vi "GPIB_SR400_A.vi"(11 "N per point":i32=1) -> (0 "A Gate":dbl[](array[numeric]), 2 "x/y":dbl)   [LabVIEW 2024]
uses:
  <vilib>/Utility/error.llb/Trim Whitespace One-Sided.vi
  GPIB_Address.vi
panel:
  out "String":string
  in  "VISA resource name":refnum<visa-resource-name>="GPIB0::23::INSTR"
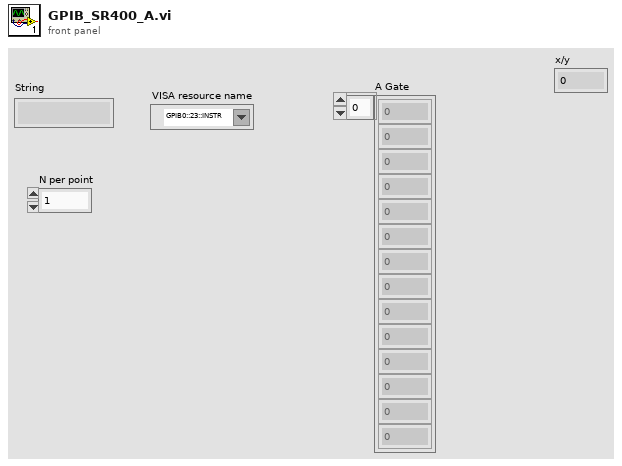
[diagram p1: front panel]
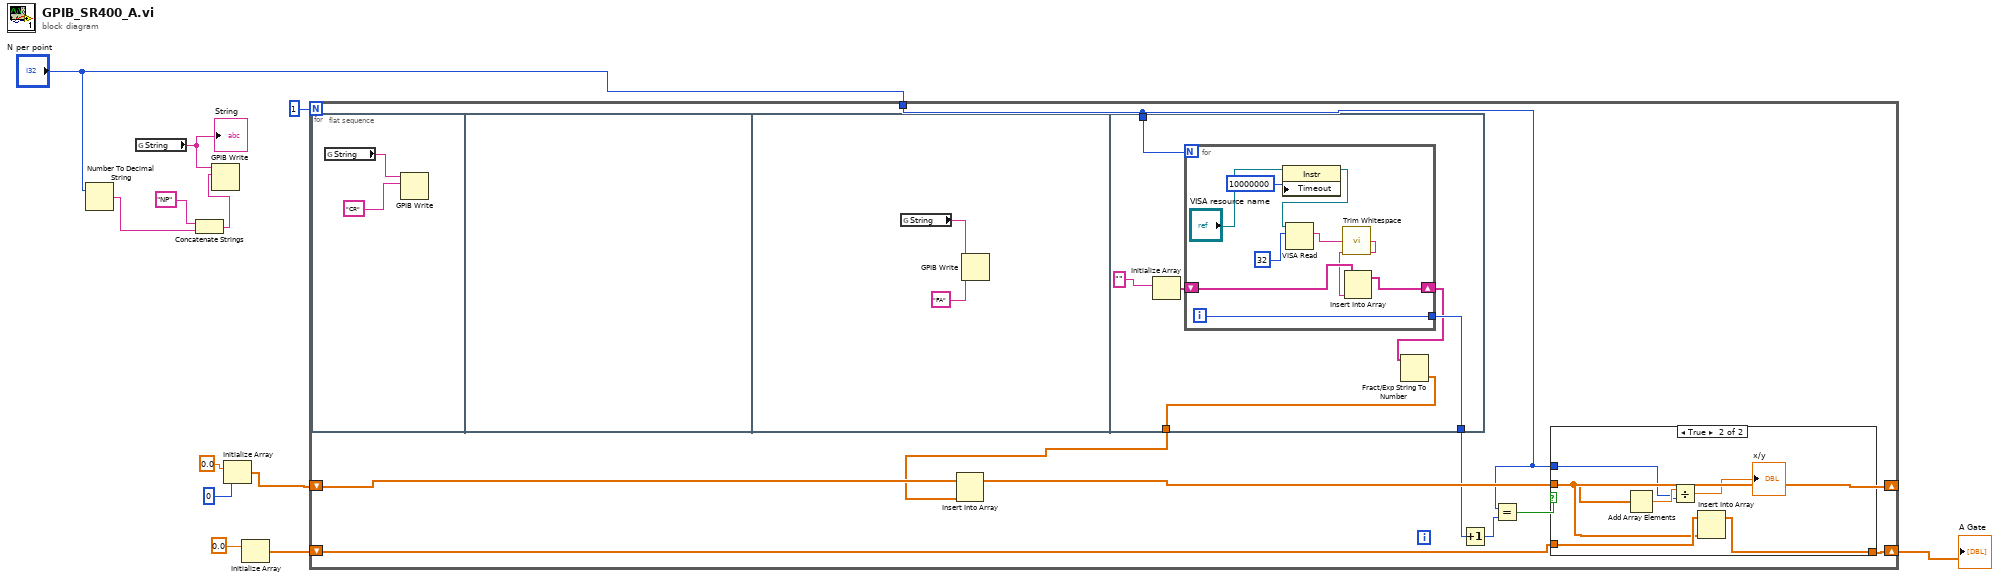
[diagram p0: block diagram]
diagram:
  n1 = Number To Decimal String(number="N per point") -> (decimal integer string=w4:string)  [unwired: 1 in]
  n2 = global read "GPIB_Address.vi" "String"() -> (w7:string)
  "String" <- w7
  n3 = Concatenate Strings("NP" ("data"), w4) -> (w3:string)
  n4 = GPIB Write(0:w7, 1:w3) -> ()  [unwired: 3 in, 2 out]
  n5 = Initialize Array(0.0, 0 ("dimension size")) -> (w12:dbl[])
  n6 = Initialize Array(0.0) -> (w10:dbl[])  [unwired: 1 in]
  n7 = for {
    N: 1 -> [_]
    shift-right: [w19] -> _
    shift-left: w12 -> [w21]
    shift-right: [w17] -> w9
    shift-left: w10 -> [w16]
    tunnel: "N per point" -> [w15]
    n8 = flat-sequence {
      tunnel: w15 -> [w37]
      tunnel: [w34] -> w14
      tunnel: [w32] -> w13
      frame #0 {
        n9 = global read "GPIB_Address.vi" "String"() -> (w28:string)
        n10 = GPIB Write(0:w28, 1:"CR" ("data")) -> ()  [unwired: 3 in, 2 out]
      }
      frame #1 {
      }
      frame #2 {
        n11 = global read "GPIB_Address.vi" "String"() -> (w30:string)
        n12 = GPIB Write(0:w30, 1:"FA" ("data")) -> ()  [unwired: 3 in, 2 out]
      }
      frame #3 {
        n13 = Initialize Array("") -> (w35:string[])  [unwired: 1 in]
        n14 = for {
          N: w37 -> [_]
          shift-right: [w44] -> w33
          shift-left: w35 -> [w45]
          tunnel: [w38] -> w34
          i -> [w38]
          n15 = property class="Instr"(reference="VISA resource name", "Timeout"=u32 10000000 ("General Settings:Timeout Value")) -> (reference out=w39:refnum<visa-resource-name>)  [unwired: 1 in, 1 out]
          n16 = VISA Read(VISA resource name=w39, byte count=32) -> (read buffer=w42:string)  [unwired: 1 in, 3 out]
          n17 = call <vilib>:"Trim Whitespace.vi"("string"=w42) -> ("trimmed string"=w43:string)  [unwired: 1 in]
          n18 = Insert Into Array "Insert Into Array"(array=w45, new element=w43) -> (w44:string[])  [unwired: 1 in]
        }
        n19 = Fract/Exp String To Number(string=w33) -> (number=w32:dbl[])  [unwired: 3 in, 1 out]
      }
    }
    n20 = Insert Into Array "Insert Into Array"(array=w21, new element=w13) -> (w19:dbl[])  [unwired: 1 in]
    n21 = Increment(x=w14) -> (x+1=w18:i32)
    n22 = Equal?(x=w15, y=w18) -> (x = y?=w20:bool)
    n23 = case shown="True" w20 {
      tunnel: w19 -> [_ w22]
      tunnel: w15 -> [_ w26]
      tunnel: [_ w23] -> w17
      tunnel: w16 -> [_ w24]
      frame False {
      }
      frame True {
        n24 = Add Array Elements(numeric array=w22) -> (sum=w27:dbl)
        n25 = Divide(x=w27, y=w26) -> (x/y=→"x/y":dbl)
        n26 = Insert Into Array(array=w24, new element=w22) -> (w23:dbl[])  [unwired: 1 in]
      }
    }
  }
  "A Gate" <- w9
